vi "R Table Graph VI.vi"(9 "R Signal Count":dbl[](array[numeric]), 10 "Region STD":dbl[](array[numeric]), 11 "Region BL":dbl[](array[numeric])) -> (1 "Count Graph":cluster{i32[], "Count":dbl[]}[](graph), 2 "STDW Graph":cluster{i32[], "Count":dbl[]}[](graph), 3 "BLW Graph":cluster{i32[], "Count":dbl[]}[](graph))   [LabVIEW 2018]
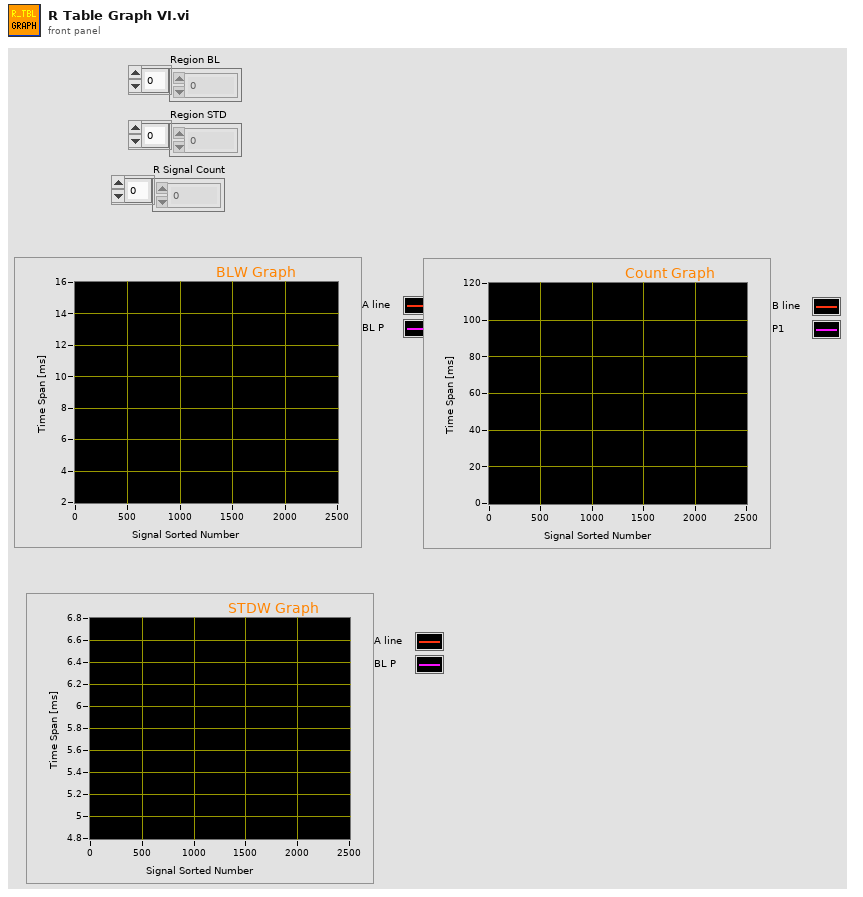
[diagram p1: front panel]
types:
  T1 = cluster{"Region BL":dbl[], "Region STD":dbl[], "R Signal Count":dbl[]}
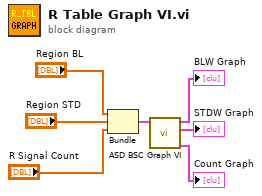
[diagram p0: block diagram]
diagram:
  n1 = Bundle("Region BL"="Region BL", "Region STD"="Region STD", "R Signal Count"="R Signal Count") -> (w7:T1)  [unwired: 1 in]
  n2 = call "ASD BSC Graph VI.vi"("Region C"=w7) -> ("Count Graph"=→"Count Graph":cluster{i32[], "Count":dbl[]}[], "STDW Graph"=→"STDW Graph":cluster{i32[], "Count":dbl[]}[], "BLW Graph"=→"BLW Graph":cluster{i32[], "Count":dbl[]}[])  [unwired: 8 in]
